vi "Converting floating point numbers_LV2014.vi"() -> ()   [LabVIEW 2014]
panel:
  in  "String (without \"Ende\")":string
  out "Fiber type at fiber port":u8[](array[numeric])
  out "Global V-T parameters":sgl[][](array[numeric]) format="%.4e"
  out "Global T-V parameters":sgl[][](array[numeric]) format="%.4e"
  out "command":string
  in  "T-V Parameter":sgl
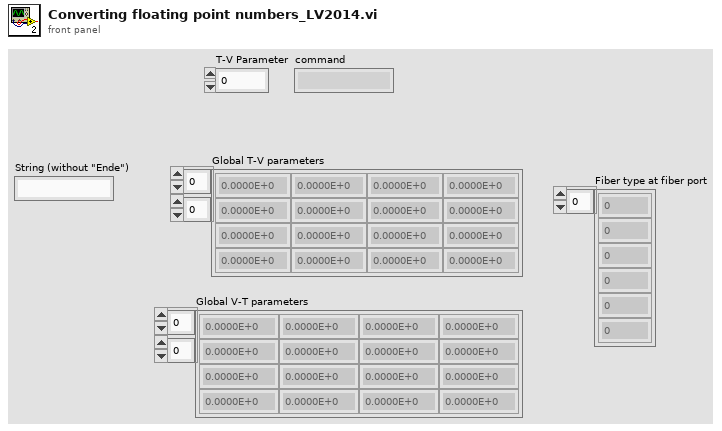
[diagram p1: front panel]
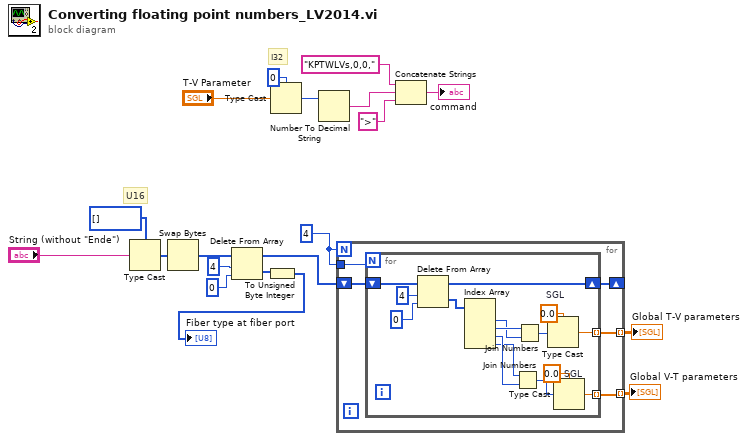
[diagram p0: block diagram]
diagram:
  w12 = 4
  # "I32"
  # "U16"
  n1 = Type Cast(type=u16[] [] ("Angehängtes Array"), x="String (without \"Ende\")") -> (*(type *) &x=w2:u16[])
  n2 = Swap Bytes(anything=w2) -> (byte swapped=w11:u16[])
  n3 = Delete From Array(array=w11, length=4 ("Länge"), index=0 ("Index")) -> (deleted portion=w6:u16[], array with subset deleted=w8:u16[])
  n4 = To Unsigned Byte Integer(number=w6) -> (unsigned 8bit integer=→"Fiber type at fiber port":u8[])
  n5 = Type Cast(type=0 ("I32"), x="T-V Parameter") -> (*(type *) &x=w19:i32)
  n6 = Number To Decimal String(number=w19) -> (decimal integer string=w14:string)  [unwired: 1 in]
  n7 = for {
    N: w12 -> [_]
    shift-right: [w23] -> _
    shift-left: w8 -> [w24]
    tunnel: [w22] -> w9 mode=indexing
    tunnel: [w21] -> w10 mode=indexing
    tunnel: w12 -> [w20]
    n8 = for {
      N: w20 -> [_]
      shift-right: [w38] -> w23
      shift-left: w24 -> [w39]
      tunnel: [w30] -> w22 mode=indexing
      tunnel: [w25] -> w21 mode=indexing
      w27 = sgl 0.0  # SGL
      w31 = sgl 0.0  # SGL
      n9 = Delete From Array(array=w39, length=4 ("Länge"), index=0 ("Index")) -> (deleted portion=w35:u16[], array with subset deleted=w38:u16[])
      n10 = Index Array(array=w35) -> (element #1=w28:u16, element #2=w29:u16, element #3=w34:u16, element #4=w33:u16)  [unwired: 4 in]
      n11 = Join Numbers(hi=w33, lo=w34) -> ((hi.lo)=w32:u32)
      n12 = Join Numbers(hi=w29, lo=w28) -> ((hi.lo)=w26:u32)
      n13 = Type Cast(type=w27, x=w26) -> (*(type *) &x=w25:sgl)
      n14 = Type Cast(type=w31, x=w32) -> (*(type *) &x=w30:sgl)
    }
  }
  "Global V-T parameters" <- w9
  "Global T-V parameters" <- w10
  n15 = Concatenate Strings("KPTWLVs,0,0," ("Schreibpuffer"), w14, ">" ("String")) -> (→"command":string)
